vi "Import from text file.vi"(8 "error in (no error)":errorcluster, 11 "File to import":path) -> (0 "error out":errorcluster, 3 "Text Translations":T1[](array[typedef]))   [LabVIEW 2019, in "Language Editor.lvlib"]
doc: "- - -\nCopyright (c) 2026, Merecs Engineering GmbH"
uses:
  Language Editor.lvlib
  Language Selection/TypeDefs/Cluster Language.ctl
  Language Selection/TypeDefs/Cluster PropertyTranslation.ctl
  Language Selection/TypeDefs/Enum Property Type.ctl
  <vilib>/Utility/file.llb/Read Delimited Spreadsheet (string).vi
  Language Selection/Language Selection.lvlib
panel:
  out "all rows":string[][](array[string])
  in  "Type (zukünftig!)":enum16{"ANSI", "Unicode"}(ring)
  # "Connector Pane"
  # "Locals"
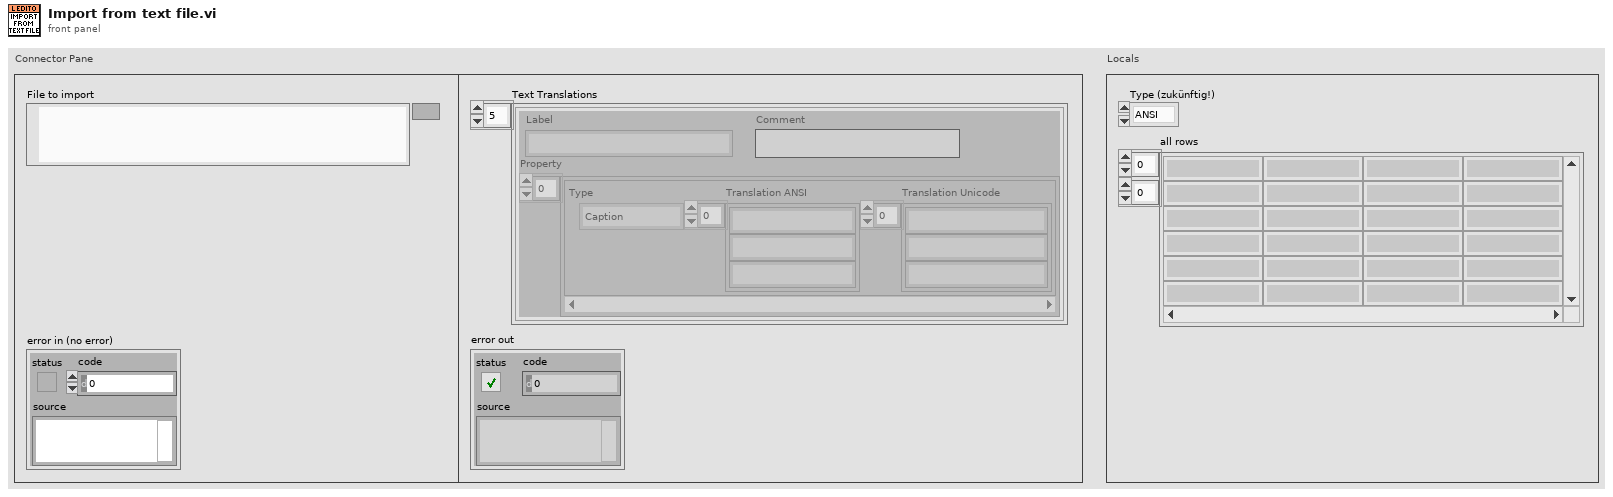
[diagram p1: front panel]
types:
  T1 = typedef "Language Selection.lvlib/Cluster Language.ctl" = cluster{"Label":string, "Comment":string, "Property":T2[]}
  T2 = typedef "Language Selection.lvlib/Cluster PropertyTranslation.ctl" = cluster{"Type":T3, "Translation ANSI":string[], "Translation Unicode":string[]}
  T3 = typedef "Language Selection.lvlib/Enum Property Type.ctl" = enum16{"NA", "Caption", "String Value", "Boolean Text", "Ring Strings", "1D Array Elements", "2D Array Elements", "(MC)Listbox Header", "(MC)Listbox Items", "Tab Pages Names", "X & Y GraphChart", "Plot Names", "Table Headers", "Table Items", "TipStrip", "Combobox Strings", "Cursor Name", "Tree Col Headers"}
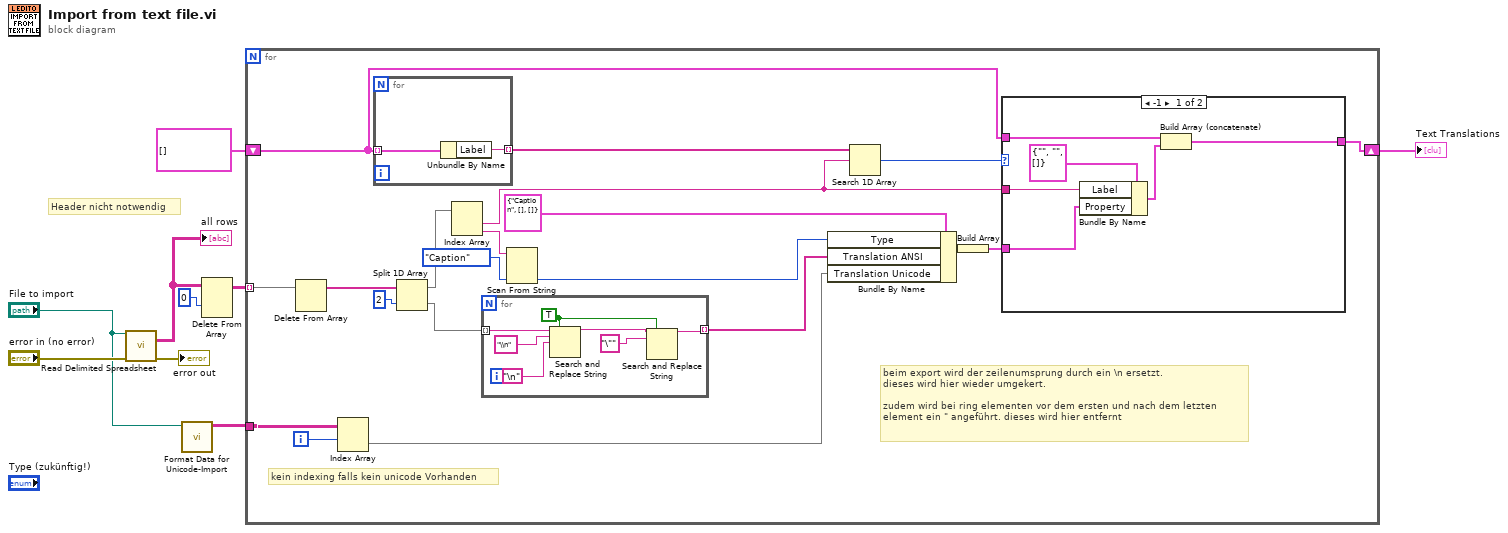
[diagram p0: block diagram]
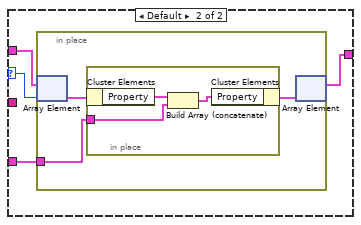
[diagram p2: hidden frame]
diagram:
  # "Header nicht notwendig"
  n1 = call-poly <vilib>:"Read Delimited Spreadsheet.vi"("file path (dialog if empty)"="File to import", "error in (no error)"="error in (no error)") -> ("all rows"=w8:string[][], "error out"=→"error out":errorcluster)  [unwired: 8 in, 4 out]
  "all rows" <- w8
  n2 = call "Format Data for Unicode-Import.vi"("file (use dialog)"="File to import") -> ("subarray"=w1:string[][])  [unwired: 10 in]
  n3 = Delete From Array(array=w8, index (row)=0) -> (array with subset deleted=w6:string[][])  [unwired: 2 in, 1 out]
  n4 = for {
    tunnel: w6 -> [w14] mode=indexing
    shift-right: [w19] -> w3
    shift-left: T1[] [] ("Translation") -> [w21]
    tunnel: w1 -> [w12]
    i -> [w11]
    # "kein indexing falls kein unicode Vorhanden"
    # "beim export wird der zeilenumsprung durch ein \\n ersetzt.\ndieses wird hier wieder umgekert.\n\nzudem wird bei ring elementen vor dem ersten und nach dem letzten\nelement ein \" angeführt. dieses wird hier entfernt"
    n5 = Delete From Array(array=w14) -> (array with subset deleted=w13:string[])  [unwired: 2 in, 1 out]
    n6 = Index Array(array=w12, index (row)=w11) -> (element=w10:string[])  [unwired: 1 in]
    n7 = for {
      tunnel: w21 -> [w54] mode=indexing
      tunnel: [w53] -> w22 mode=indexing
      n8 = Unbundle By Name(w54) -> ("Label"=w53:string)
    }
    n9 = Split 1D Array(array=w13, index=2) -> (first subarray=w26:string[], second subarray=w16:string[])
    n10 = Index Array(array=w26) -> (element #1=w18:string, element #2=w28:string)  [unwired: 2 in]
    n11 = for {
      tunnel: w16 -> [w35] mode=indexing
      tunnel: [w33] -> w15 mode=indexing
      w31 = TRUE ("replace all? (F)")
      n12 = Search and Replace String(replace all?=w31, input string=w35, search string="\\n", replace string="\n") -> (result string=w32:string)  [unwired: 4 in, 3 out]
      n13 = Search and Replace String(replace all?=w31, input string=w32, search string="\"") -> (result string=w33:string)  [unwired: 5 in, 3 out]
    }
    n14 = Scan From String(input string=w28, default 1=Enum_Property_Type."Caption" ("Type")) -> (output 1=w27:T3)  [unwired: 3 in, 3 out]
    n15 = Bundle By Name(cluster=T2 {"Type"=enum."Caption", "Translation ANSI"=[], "Translation Unicode"=[]} ("Obj."), "Type"=w27, "Translation ANSI"=w15, "Translation Unicode"=w10) -> (w24:T2)
    n16 = Search 1D Array(1D array=w22, element=w18) -> (index of element=w20:i32)  [unwired: 1 in]
    n17 = Build Array(w24) -> (w17:T2[])
    n18 = case shown="-1" w20 {
      selector: w20 -> [_ w45]
      tunnel: w21 -> [w40 w46]
      tunnel: w17 -> [w37 w44]
      tunnel: [w39 w43] -> w19
      tunnel: w18 -> [w42 _]
      frame -1 {
        n19 = Bundle By Name(cluster=T1 {"Label"="", "Comment"="", "Property"=[]} ("Translation"), "Label"=w42, "Property"=w37) -> (w38:T1)
        n20 = Build Array (concatenate)(w40, w38) -> (w39:T1[])
      }
      frame Default {
        n21 = in-place {
          in-place-border: w44 -> [w48]
          n22 = in-place-array #1(w46, w45) -> (w49:T1)
          n23 = in-place {
            in-place-border: w48 -> [w50]
            n24 = in-place-cluster #2(w49) -> ("Property"=w52:T2[])
            n25 = Build Array (concatenate)(w52, w50) -> (w51:T2[])
            n26 = in-place-cluster #2("Property"=w51) -> (w47:T1)
          }
          n27 = in-place-array #1(w47) -> (w43:T1[])  [unwired: 1 out]
        }
      }
    }
  }
  "Text Translations" <- w3
